vi "Write Relay.vi"(8 "error in (no error)":errorcluster, 9 "Relay (1 based)":u8, 10 "On / Off":bool, 11 "Device":string="hidraw0") -> (0 "error out":errorcluster)   [LabVIEW 2021, in "USB Relay Control.lvlib"]
uses:
  typedef/Read Write.ctl
  USB Relay Control.lvlib
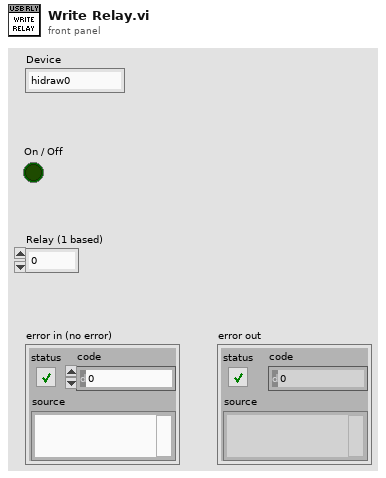
[diagram p1: front panel]
types:
  T1 = typedef "USB Relay Control.lvlib/Read Write.ctl" = enum8{"Read", "Write"}
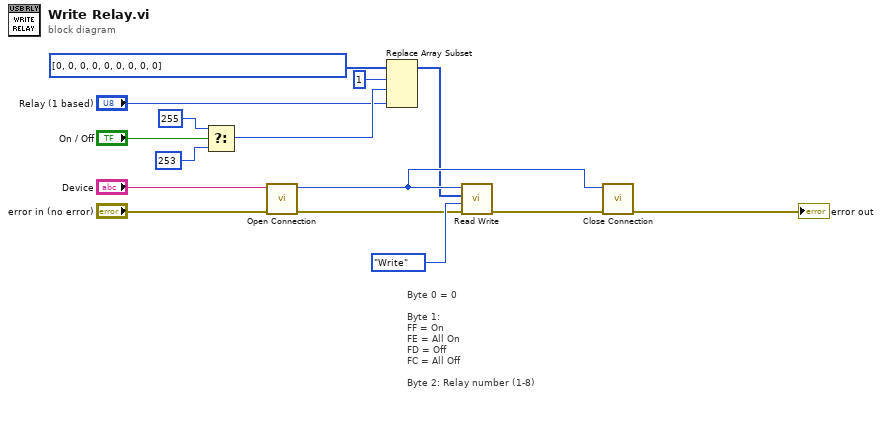
[diagram p0: block diagram]
diagram:
  # "Byte 0 = 0\n\nByte 1:\nFF = On\nFE = All On\nFD = Off\nFC = All Off\n\nByte 2: Relay number (1-8)"
  n1 = Select(t=u8 255, s="On / Off", f=u8 253) -> (s? t:f=w2:u8)
  n2 = call "Open Connection.vi"("error in (no error)"="error in (no error)", "Device"="Device") -> ("error out"=w12:errorcluster, "HID RAW Reference"=w14:i32)  [unwired: 8 in]
  n3 = Replace Array Subset(array=u8[] [0, 0, 0, 0, 0, 0, 0, 0, 0] ("Buffer In"), new element #1=w2, index #1=1 ("index"), new element #2="Relay (1 based)") -> (w9:u8[])  [unwired: 1 in]
  n4 = call "Read Write.vi"("error in (no error)"=w12, "RW"=Read_Write."Write", "Buffer In"=w9, "HID RAW Reference"=w14) -> ("error out"=w6:errorcluster)  [unwired: 6 in, 1 out]
  n5 = call "Close Connection.vi"("error in (no error)"=w6, "HID RAW Reference"=w14) -> ("error out"=→"error out":errorcluster)  [unwired: 9 in]
